vi "Test CIF pcap PubSub Raw.vi"() -> ()   [LabVIEW 2021]
uses:
  Iceoryx.lvlib
  typedef/CIF Pcap Publisher Configuration.ctl
  typedef/CIF Pcap Subscriber Configuration.ctl
  typedef/CIF Channel Header Publisher.ctl
  typedef/CIF Channel Header.ctl
panel:
  out "status":string
  out "pass":bool
  out "error out":errorcluster
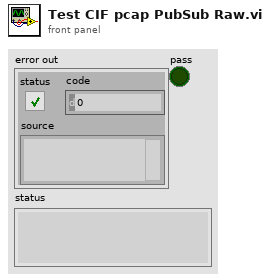
[diagram p1: front panel]
types:
  T1 = typedef "Iceoryx.lvlib/CIF Channel Header Publisher.ctl" = cluster{"T0":i64, "T_Out":i64, "T_Tx":i64, "ClockID":u8}
  T2 = typedef "Iceoryx.lvlib/CIF Pcap Subscriber Configuration.ctl" = cluster{"Name":string, "Topic":string, "Link Type":u32, "Backpressure":bool}
  T3 = typedef "Iceoryx.lvlib/CIF Pcap Publisher Configuration.ctl" = cluster{"Name":string, "Topic":string, "Link Type":u32, "Descriptor":string, "Max Bytes":u32, "Best Effort Subscribers":u32, "Backpressure Subscribers":u32, "Best Effort Queue Depth":u32, "Backpressure Queue Depth":u32}
  T4 = typedef "Iceoryx.lvlib/CIF Channel Header.ctl" = cluster{"Length":u64, "T0":i64, "T_Out":i64, "T_Tx":i64, "Ctr":u64, "ClockID":u8}
  T5 = typedef "Iceoryx.lvlib/CIF Publisher Refnum.ctl" = cluster{"refnum":u64, "CIF Pub":enum8{"cifpub"}}
  T6 = typedef "Iceoryx.lvlib/CIF Subscriber Refnum.ctl" = cluster{"refnum":u64, "CIF Sub":enum8{"cifsub"}}
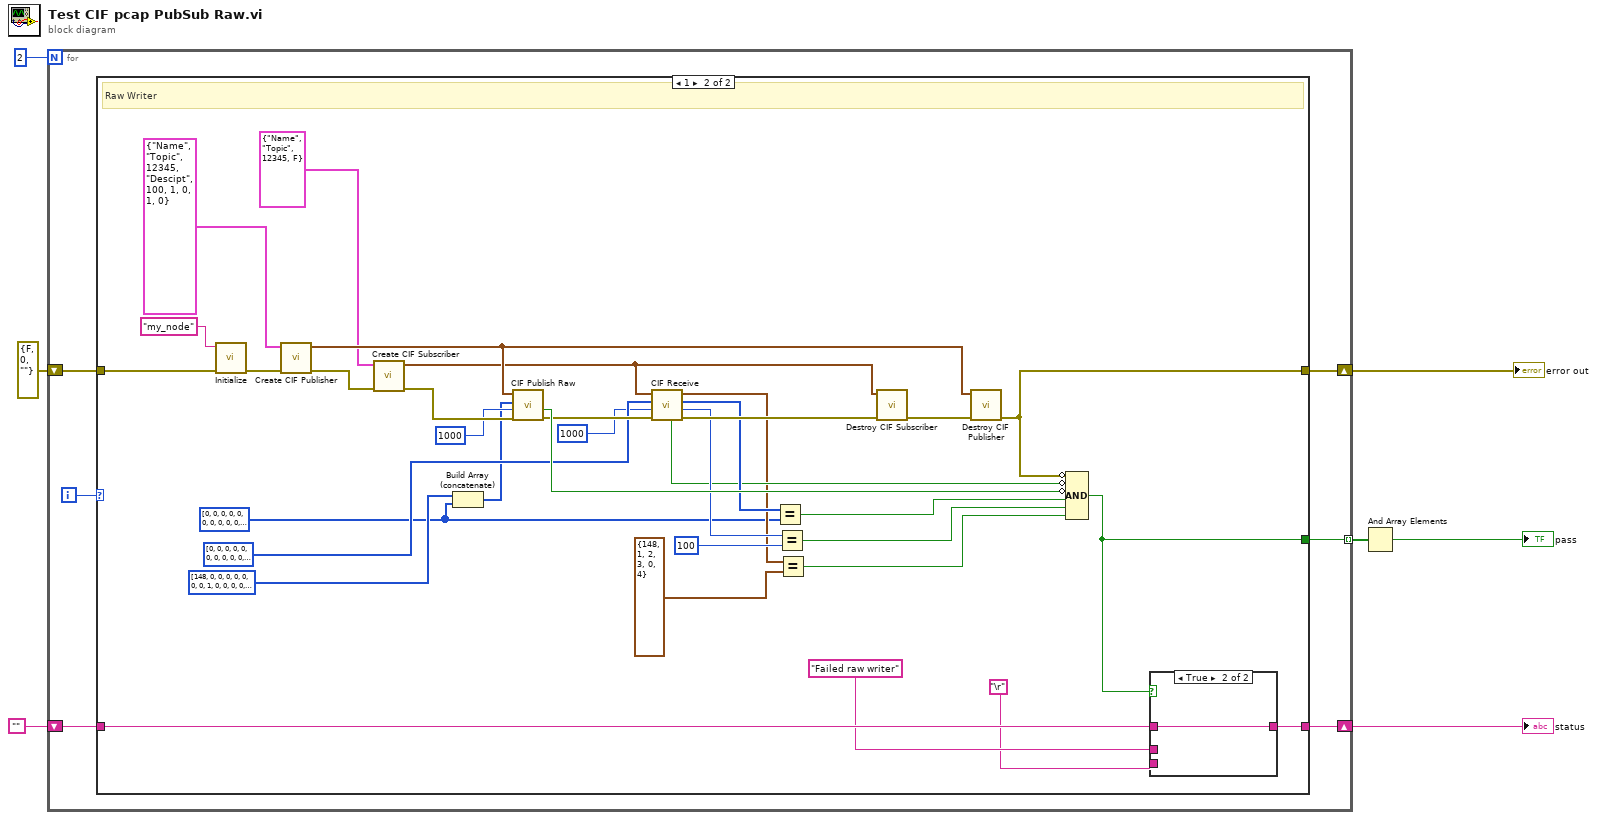
[diagram p0: block diagram]
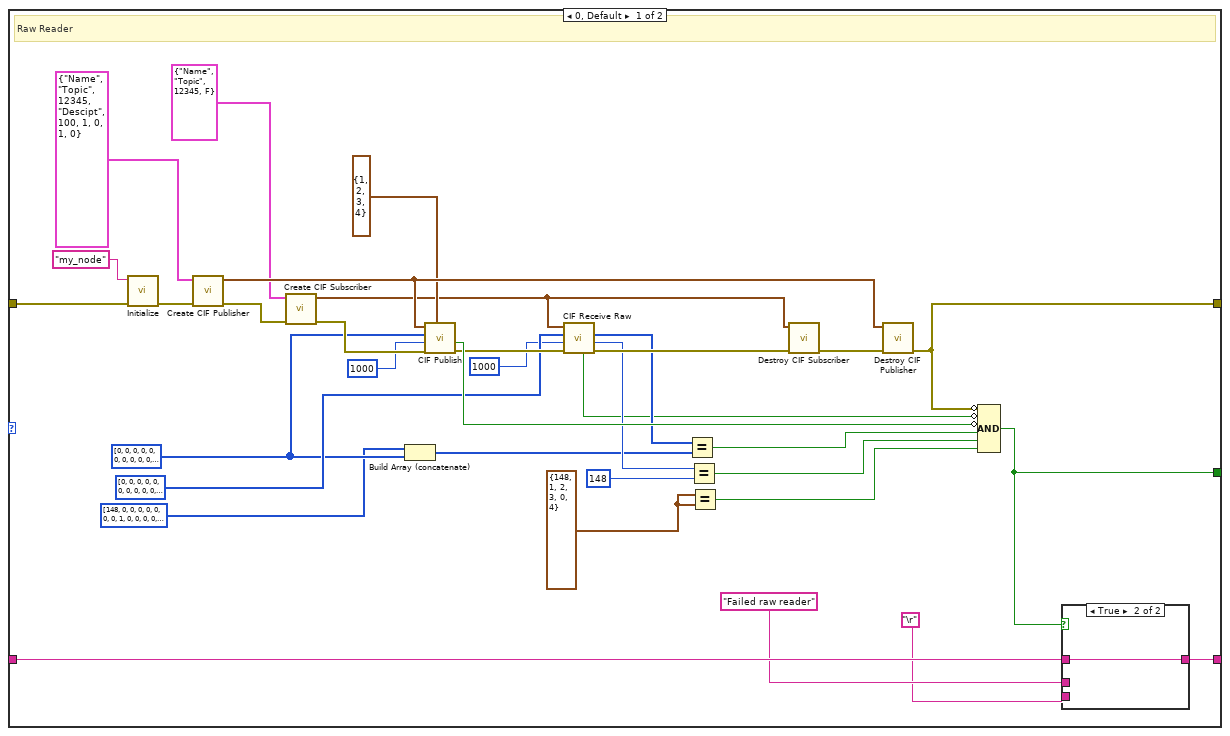
[diagram p2: hidden frame]
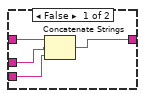
[diagram p3: hidden frame]
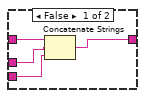
[diagram p4: hidden frame]
diagram:
  n1 = for {
    N: 2 -> [_]
    tunnel: [w13] -> w7 mode=indexing
    shift-right: [w10] -> w3
    shift-left: "" -> [w11]
    shift-right: [w9] -> w1
    shift-left: errorcluster {"status"=FALSE, "code"=0, "source"=""} ("error out") -> [w8]
    i -> [w12]
    n2 = case shown="1" w12 {
      tunnel: [w43 w82] -> w13
      tunnel: w11 -> [w47 w86]
      tunnel: [w46 w85] -> w10
      tunnel: [w35 w74] -> w9
      tunnel: w8 -> [w42 w81]
      frame 0, Default {
        w17 = T4 {"Length"=148, "T0"=1, "T_Out"=2, "T_Tx"=3, "Ctr"=0, "ClockID"=4} ("CIF Channel Header")
        w16 = u8[] [0, 0, 0, 0, 0, 0, 0, 0, 0, 0, 0, 0, 0, 0, 0, 0, 0, 0, 0, 0, 0, 0, 0, 0, 0, 0, 0, 0, 0, 0, 0, 0, 0, 0, 0, 0, 0, 0, 0, 0, 0, 0, 0, 0, 0, 0, 0, 0, 0, 0, 0, 0, 0, 0, 0, 0, 0, 0, 0, 0, 0, 0, 0, 0, 0, 0, 0, 0, 0, 0, 0, 0, 0, 0, 0, 0, 0, 0, 0, 0, 0, 0, 0, 0, 0, 0, 0, 0, 0, 0, 0, 0, 0, 0, 0, 0, 0, 0, 0, 1] ("Data In")
        # "Raw Reader"
        n3 = call "Initialize.vi"("error in (no error)"=w42, "Node name"="my_node") -> ("error out"=w40:errorcluster)  [unwired: 9 in]
        n4 = call "Create CIF Publisher.vi"("error in (no error)"=w40, "CIF Pcap Publisher Configuration"=T3 {"Name"="Name", "Topic"="Topic", "Link Type"=12345, "Descriptor"="Descipt", "Max Bytes"=100, "Best Effort Subscribers"=1, "Backpressure Subscribers"=0, "Best Effort Queue Depth"=1, "Backpressure Queue Depth"=0}) -> ("error out"=w39:errorcluster, "CIF Publisher Refnum"=w36:T5)  [unwired: 8 in]
        n5 = call "Create CIF Subscriber.vi"("error in (no error)"=w39, "CIF Pcap Subscriber Configuration"=T2 {"Name"="Name", "Topic"="Topic", "Link Type"=12345, "Backpressure"=FALSE}) -> ("error out"=w38:errorcluster, "CIF Subscriber Refnum"=w25:T6)  [unwired: 8 in]
        n6 = Build Array (concatenate)(u8[] [148, 0, 0, 0, 0, 0, 0, 0, 1, 0, 0, 0, 0, 0, 0, 0, 2, 0, 0, 0, 0, 0, 0, 0, 3, 0, 0, 0, 0, 0, 0, 0, 0, 0, 0, 0, 0, 0, 0, 0, 4, 0, 0, 0, 0, 0, 0, 0] ("Data In"), w16) -> (w14:u8[])
        n7 = call "CIF Publish.vi"("CIF Channel Header Publisher"=T1 {"T0"=1, "T_Out"=2, "T_Tx"=3, "ClockID"=4}, "error in (no error)"=w38, "Timeout ms"=u32 1000 ("Timoeut ms"), "Data In"=w16, "Publisher Reference"=w36) -> ("error out"=w24:errorcluster, "Timeout"=w32:bool)  [unwired: 3 in, 2 out]
        n8 = call "CIF Receive Raw.vi"("error in (no error)"=w24, "Timoeut ms"=u32 1000, "Data In"=u8[] [0, 0, 0, 0, 0, 0, 0, 0, 0, 0, 0, 0, 0, 0, 0, 0, 0, 0, 0, 0, 0, 0, 0, 0, 0, 0, 0, 0, 0, 0, 0, 0, 0, 0, 0, 0, 0, 0, 0, 0, 0, 0, 0, 0, 0, 0, 0, 0, 0, 0, 0, 0, 0, 0, 0, 0, 0, 0, 0, 0, 0, 0, 0, 0, 0, 0, 0, 0, 0, 0, 0, 0, 0, 0, 0, 0, 0, 0, 0, 0, 0, 0, 0, 0, 0, 0, 0, 0, 0, 0, 0, 0, 0, 0, 0, 0, 0, 0, 0, 0, 0, 0, 0, 0, 0, 0, 0, 0, 0, 0, 0, 0, 0, 0, 0, 0, 0, 0, 0, 0, 0, 0, 0, 0, 0, 0, 0, 0, 0, 0, 0, 0, 0, 0, 0, 0, 0, 0, 0, 0, 0, 0, 0, 0, 0, 0, 0, 0], "Subscriber Reference"=w25) -> ("error out"=w23:errorcluster, "Array Length"=w21:u32, "Data Out"=w20:u8[], "Timeout"=w19:bool)  [unwired: 3 in, 1 out]
        n9 = Equal?(x=w20, y=w14) -> (x = y?=w33:bool)
        n10 = Equal?(x=w21, y=u32 148) -> (x = y?=w27:bool)
        n11 = Equal?(x=w17, y=w17) -> (x = y?=w26:bool)
        n12 = call "Destroy CIF Subscriber.vi"("error in (no error)"=w23, "Subscriber Reference"=w25) -> ("error out"=w37:errorcluster)  [unwired: 9 in]
        n13 = call "Destroy CIF Publisher.vi"("error in (no error)"=w37, "Publisher Reference"=w36) -> ("error out"=w35:errorcluster)  [unwired: 9 in]
        n14 = Compound Arithmetic op=AND(invert w35, invert w19, invert w32, w33, w27, w26) -> (w43:bool)
        n15 = case shown="True" w43 {
          tunnel: w47 -> [w51 w52]
          tunnel: [w48 w52] -> w46
          tunnel: "Failed raw reader" -> [w50 _]
          tunnel: "\r" -> [w49 _]
          frame False {
            n16 = Concatenate Strings(w51, w50, w49) -> (w48:string)
          }
          frame True {
          }
        }
      }
      frame 1 {
        w53 = u8[] [0, 0, 0, 0, 0, 0, 0, 0, 0, 0, 0, 0, 0, 0, 0, 0, 0, 0, 0, 0, 0, 0, 0, 0, 0, 0, 0, 0, 0, 0, 0, 0, 0, 0, 0, 0, 0, 0, 0, 0, 0, 0, 0, 0, 0, 0, 0, 0, 0, 0, 0, 0, 0, 0, 0, 0, 0, 0, 0, 0, 0, 0, 0, 0, 0, 0, 0, 0, 0, 0, 0, 0, 0, 0, 0, 0, 0, 0, 0, 0, 0, 0, 0, 0, 0, 0, 0, 0, 0, 0, 0, 0, 0, 0, 0, 0, 0, 0, 0, 1] ("Data In")
        # "Raw Writer"
        n17 = call "Initialize.vi"("error in (no error)"=w81, "Node name"="my_node") -> ("error out"=w79:errorcluster)  [unwired: 9 in]
        n18 = call "Create CIF Publisher.vi"("error in (no error)"=w79, "CIF Pcap Publisher Configuration"=T3 {"Name"="Name", "Topic"="Topic", "Link Type"=12345, "Descriptor"="Descipt", "Max Bytes"=100, "Best Effort Subscribers"=1, "Backpressure Subscribers"=0, "Best Effort Queue Depth"=1, "Backpressure Queue Depth"=0}) -> ("error out"=w78:errorcluster, "CIF Publisher Refnum"=w75:T5)  [unwired: 8 in]
        n19 = call "Create CIF Subscriber.vi"("error in (no error)"=w78, "CIF Pcap Subscriber Configuration"=T2 {"Name"="Name", "Topic"="Topic", "Link Type"=12345, "Backpressure"=FALSE}) -> ("error out"=w77:errorcluster, "CIF Subscriber Refnum"=w65:T6)  [unwired: 8 in]
        n20 = Build Array (concatenate)(u8[] [148, 0, 0, 0, 0, 0, 0, 0, 1, 0, 0, 0, 0, 0, 0, 0, 2, 0, 0, 0, 0, 0, 0, 0, 3, 0, 0, 0, 0, 0, 0, 0, 0, 0, 0, 0, 0, 0, 0, 0, 4, 0, 0, 0, 0, 0, 0, 0] ("Data In"), w53) -> (w54:u8[])
        n21 = call "CIF Publish Raw.vi"("error in (no error)"=w77, "Timoeut ms"=u32 1000, "Data In"=w54, "Publisher Reference"=w75) -> ("error out"=w64:errorcluster, "Timeout"=w71:bool)  [unwired: 4 in, 2 out]
        n22 = call "CIF Receive.vi"("error in (no error)"=w64, "Timoeut ms"=u32 1000, "Data In"=u8[] [0, 0, 0, 0, 0, 0, 0, 0, 0, 0, 0, 0, 0, 0, 0, 0, 0, 0, 0, 0, 0, 0, 0, 0, 0, 0, 0, 0, 0, 0, 0, 0, 0, 0, 0, 0, 0, 0, 0, 0, 0, 0, 0, 0, 0, 0, 0, 0, 0, 0, 0, 0, 0, 0, 0, 0, 0, 0, 0, 0, 0, 0, 0, 0, 0, 0, 0, 0, 0, 0, 0, 0, 0, 0, 0, 0, 0, 0, 0, 0, 0, 0, 0, 0, 0, 0, 0, 0, 0, 0, 0, 0, 0, 0, 0, 0, 0, 0, 0, 0], "Subscriber Reference"=w65) -> ("error out"=w63:errorcluster, "Array Length"=w61:u32, "Data Out"=w60:u8[], "CIF Channel Header"=w55:T4, "Timeout"=w59:bool)  [unwired: 2 in, 1 out]
        n23 = Equal?(x=w60, y=w53) -> (x = y?=w72:bool)
        n24 = Equal?(x=w61, y=u32 100) -> (x = y?=w67:bool)
        n25 = Equal?(x=w55, y=T4 {"Length"=148, "T0"=1, "T_Out"=2, "T_Tx"=3, "Ctr"=0, "ClockID"=4} ("CIF Channel Header")) -> (x = y?=w66:bool)
        n26 = call "Destroy CIF Subscriber.vi"("error in (no error)"=w63, "Subscriber Reference"=w65) -> ("error out"=w76:errorcluster)  [unwired: 9 in]
        n27 = call "Destroy CIF Publisher.vi"("error in (no error)"=w76, "Publisher Reference"=w75) -> ("error out"=w74:errorcluster)  [unwired: 9 in]
        n28 = Compound Arithmetic op=AND(invert w74, invert w59, invert w71, w72, w67, w66) -> (w82:bool)
        n29 = case shown="True" w82 {
          tunnel: w86 -> [w90 w91]
          tunnel: [w87 w91] -> w85
          tunnel: "Failed raw writer" -> [w89 _]
          tunnel: "\r" -> [w88 _]
          frame False {
            n30 = Concatenate Strings(w90, w89, w88) -> (w87:string)
          }
          frame True {
          }
        }
      }
    }
  }
  "error out" <- w1
  "status" <- w3
  n31 = And Array Elements(Boolean array=w7) -> (logical AND=→"pass":bool)
